vi "layout.vi"(0 "reference":refnum<class "SystemNode.lvclass">, 1 "graph":refnum<class "Graph.lvclass">, 2 "graphics":refnum<class "Graphics.lvclass">, 3 "grid":refnum<class "Grid.lvclass">, 5 "error in (no error)":errorcluster) -> (14 "reference out":refnum<class "SystemNode.lvclass">, 19 "error out":errorcluster)   [LabVIEW 2020, in "SystemNode.lvclass"]
doc: "public void draw(Graphics2D g2)"
uses:
  <resource>/Framework/Providers/Open_GDS/UML/SystemNode_class/SystemNode.lvclass
  C:/Program Files (x86)/National Instruments/LabVIEW 2020/resource/Framework/Providers/Open_GDS/UML/RectangularNode_class/RectangularNode.lvclass
  C:/Program Files (x86)/National Instruments/LabVIEW 2020/resource/Framework/Providers/Open_GDS/UML/AbstractNode_class/AbstractNode.lvclass
  <resource>/Framework/Providers/Open_GDS/UML/Grid_class/Grid.lvclass
  <resource>/Framework/Providers/Open_GDS/UML/Graphics_class/Graphics.lvclass
  <resource>/Framework/Providers/Open_GDS/UML/Graph_class/Graph.lvclass
  <resource>/Framework/Providers/Open_GDS/UML/General/Rectangle/Rectangle Rectangle2D.ctl
  <resource>/Framework/Providers/Open_GDS/UML/MultiLineString_class/MultiLineString.lvclass
  <resource>/Framework/Providers/Open_GDS/UML/AbstractNode_class/AbstractNode.lvclass
  <resource>/Framework/Providers/Open_GDS/UML/RectangularNode_class/RectangularNode.lvclass
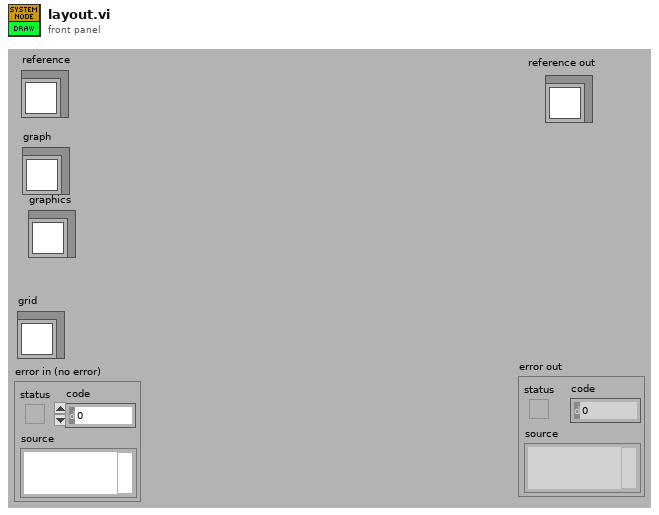
[diagram p1: front panel]
types:
  T1 = typedef "Rectangle Rectangle2D.ctl" = cluster{"x":dbl, "y":dbl, "width":dbl, "height":dbl}
  T2 = typedef "SystemNode.lvclass/ObjectAttributes.ctl" = cluster{"contents":refnum<class "MultiLineString.lvclass">, "DEFAULT_WIDTH":i32, "DEFAULT_HEIGHT":i32, "NAME_GAP":i32, "XGAP":i32, "YGAP":i32}
  T3 = typedef "RectangularNode.lvclass/ObjectAttributes.ctl" = cluster{"bounds":T1}
  T4 = typedef "AbstractNode.lvclass/ObjectAttributes.ctl" = cluster{"parent":refnum<class "AbstractNode.lvclass">, "children":refnum<class "AbstractNode.lvclass">[], "Hidden":bool}
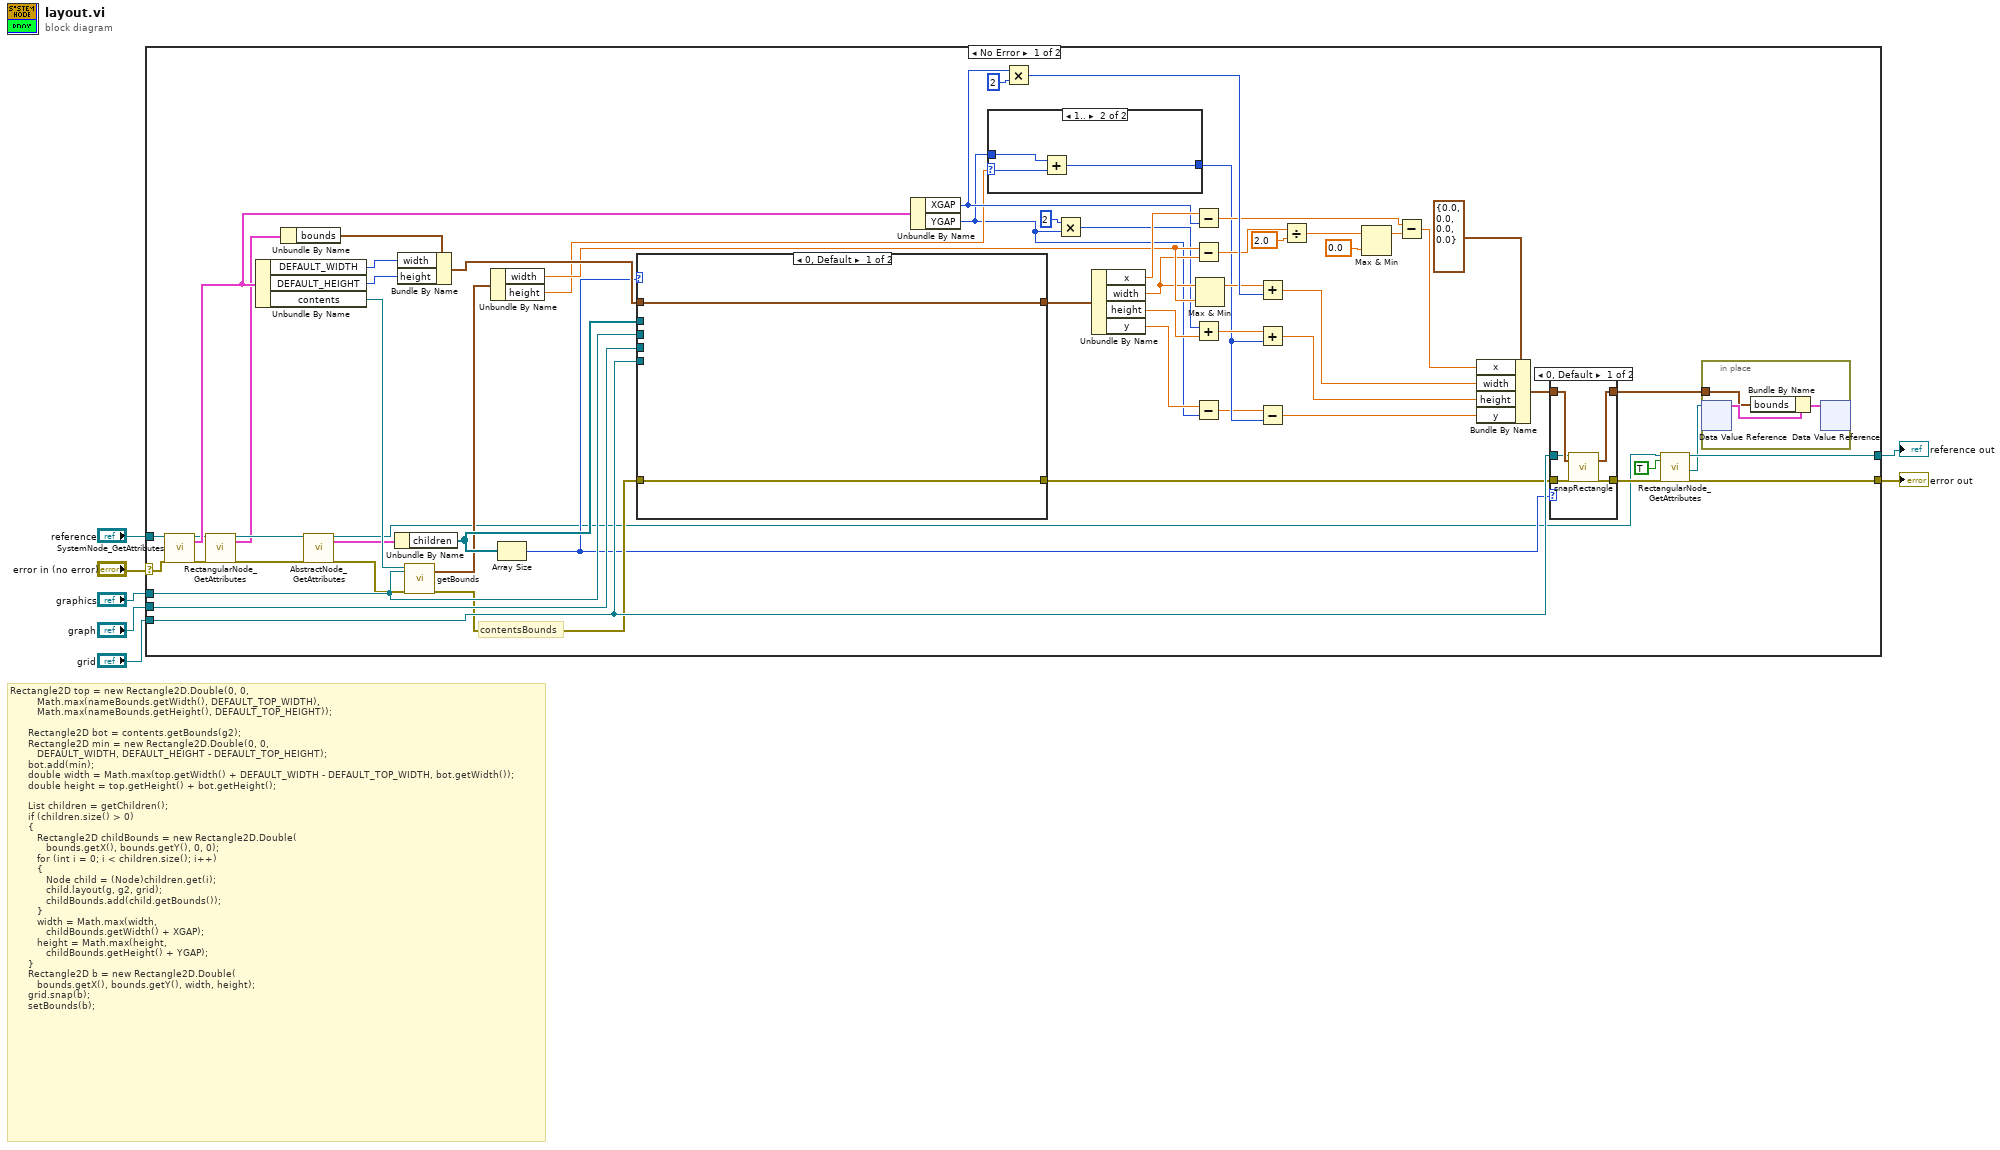
[diagram p0: block diagram]
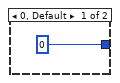
[diagram p3: hidden frame]
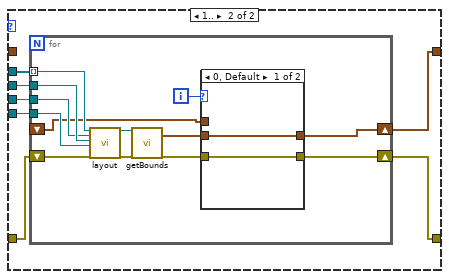
[diagram p4: hidden frame]
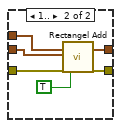
[diagram p5: hidden frame]
diagram:
  # "Rectangle2D top = new Rectangle2D.Double(0, 0,\n         Math.max(nameBounds.getWidth(), DEFAULT_TOP_WIDTH), \n         Math.max(nameBounds.getHeight(), DEFAULT_TOP_HEIGHT));\n\n      Rectangle2D bot = contents.getBounds(g2);\n      Rectangle2D min = new Rectangle2D.Double(0, 0,\n         DEFAULT_WIDTH, DEFAULT_HEIGHT - DEFAULT_TOP_HEIGHT);\n      bot.add(min);\n      double width = Math.max(top.getWidth() + DEFAULT_WIDTH - DEFAULT_TOP_WIDTH, bot.getWidth());\n      double height = top.getHeight() + bot.getHeight();\n\n      List children = getChildren();\n      if (children.size() > 0)\n      {\n         Rectangle2D childBounds = new Rectangle2D.Double(\n            bounds.getX(), bounds.getY(), 0, 0);\n         for (int i = 0; i < children.size(); i++)\n         {\n            Node child = (Node)children.get(i);\n            child.layout(g, g2, grid);\n            childBounds.add(child.getBounds());\n         }\n         width = Math.max(width, \n            childBounds.getWidth() + XGAP);\n         height = Math.max(height, \n            childBounds.getHeight() + YGAP);\n      }\n      Rectangle2D b = new Rectangle2D.Double(\n         bounds.getX(), bounds.getY(), width, height);\n      grid.snap(b);\n      setBounds(b);"
  n1 = case shown="No Error" "error in (no error)" {
    selector: "error in (no error)" -> [w63 w111]
    tunnel: "reference" -> [w66 w112]
    tunnel: [w65 w111] -> w6
    tunnel: [w64 w112] -> w5
    tunnel: "graphics" -> [w62 _]
    tunnel: "grid" -> [w61 _]
    tunnel: "graph" -> [w60 _]
    frame No Error {
      # "contentsBounds"
      n2 = call <resource>:"SystemNode_GetAttributes.vi"("reference in"=w66, "error in (no error)"=w63) -> ("reference out"=w17:refnum<class "SystemNode.lvclass">, "Data"=w18:T2, "error out"=w16:errorcluster)  [unwired: 1 in, 14 out]
      n3 = call <resource>:"RectangularNode_GetAttributes.vi"("reference in"=w17, "error in (no error)"=w16) -> ("reference out"=w15:refnum<class "SystemNode.lvclass">, "Data"=w10:T3, "error out"=w14:errorcluster)  [unwired: 14 in, 1 out]
      n4 = Unbundle By Name(w18) -> ("DEFAULT_WIDTH"=w56:i32, "DEFAULT_HEIGHT"=w57:i32, "contents"=w59:refnum<class "MultiLineString.lvclass">)
      n5 = Unbundle By Name(w10) -> ("bounds"=w55:T1)
      n6 = call <resource>:"AbstractNode_GetAttributes.vi"("reference in"=w15, "error in (no error)"=w14) -> ("reference out"=w12:refnum<class "SystemNode.lvclass">, "Data"=w11:T4, "error out"=w13:errorcluster)  [unwired: 14 in, 1 out]
      n7 = Unbundle By Name(w11) -> ("children"=w58:refnum<class "AbstractNode.lvclass">[])
      n8 = Bundle By Name(cluster=w55, "width"=w56, "height"=w57) -> (w53:T1)
      n9 = call-dynamic "getBounds.vi"("reference"=w59, "graphics"=w62, "error in (no error)"=w13) -> ("bounds"=w45:T1, "error out"=w54:errorcluster)  [unwired: 14 in, 1 out]
      n10 = Unbundle By Name(w45) -> ("width"=w43:dbl, "height"=w28:dbl)
      n11 = Array Size(array=w58) -> (size(s)=w20:i32)
      n12 = case shown="0, Default" w20 {
        tunnel: w54 -> [w82 w89]
        tunnel: w58 -> [_ w88]
        tunnel: w53 -> [w81 _]
        tunnel: [w82 w83] -> w21
        tunnel: w61 -> [_ w87]
        tunnel: w62 -> [_ w86]
        tunnel: w60 -> [_ w85]
        tunnel: [w81 w84] -> w50
        frame 0, Default {
        }
        frame 1.. {
          n13 = for {
            tunnel: w88 -> [w100] mode=indexing
            shift-right: [w102] -> w83
            shift-left: w89 -> [w101]
            shift-right: [w96] -> w84
            shift-left: _ -> [w92]
            tunnel: w87 -> [w95]
            tunnel: w86 -> [w94]
            tunnel: w85 -> [w93]
            i -> [w90]
            n14 = call-dynamic "layout.vi"("reference"=w100, "graph"=w93, "graphics"=w94, "grid"=w95, "error in (no error)"=w101) -> ("reference out"=w99:refnum<class "AbstractNode.lvclass">, "error out"=w98:errorcluster)  [unwired: 13 in]
            n15 = call-dynamic "getBounds.vi"("reference"=w99, "error in (no error)"=w98) -> ("bounds"=w91:T1, "error out"=w97:errorcluster)  [unwired: 15 in, 1 out]
            n16 = case shown="0, Default" w90 {
              tunnel: [w104 w110] -> w102
              tunnel: w97 -> [w104 w109]
              tunnel: [w103 w108] -> w96
              tunnel: w92 -> [_ w107]
              tunnel: w91 -> [w103 w106]
              frame 0, Default {
              }
              frame 1.. {
                n17 = call <resource>:"Rectangel Add.vi"("bounds1"=w107, "bounds2"=w106, "error in (no error)"=w109, "useAbsoluteCordinates(False)"=TRUE) -> ("boundsAdded"=w108:T1, "error out"=w110:errorcluster)  [unwired: 1 in, 13 out]
              }
            }
          }
        }
      }
      n18 = Unbundle By Name(w18) -> ("XGAP"=w46:i32, "YGAP"=w24:i32)
      n19 = case shown="1.." w28 {
        selector: w28 -> [_ w80]
        tunnel: w24 -> [_ w79]
        tunnel: [0 w78] -> w27
        frame 0, Default {
        }
        frame 1.. {
          n20 = Add(x=w79, y=w80) -> (x+y=w78:i32)
        }
      }
      n21 = Multiply(x=w46, y=2) -> (x*y=w48:i32)
      n22 = Multiply(x=2, y=w24) -> (x*y=w32:i32)
      n23 = Unbundle By Name(w50) -> ("x"=w49:dbl, "width"=w42:dbl, "height"=w33:dbl, "y"=w25:dbl)
      n24 = Subtract(x=w49, y=w46) -> (x-y=w40:dbl)
      n25 = Subtract(x=w43, y=w42) -> (x-y=w39:dbl)
      n26 = Add(x=w32, y=w33) -> (x+y=w30:dbl)
      n27 = Subtract(x=w25, y=w24) -> (x-y=w26:dbl)
      n28 = Max & Min(x=w42, y=w43) -> (max(x,y)=w44:dbl)  [unwired: 1 out]
      n29 = Add(x=w44, y=w48) -> (x+y=w47:dbl)
      n30 = Add(x=w30, y=w27) -> (x+y=w29:dbl)
      n31 = Subtract(x=w26, y=w27) -> (x-y=w34:dbl)
      n32 = Divide(x=w39, y=2.0) -> (x/y=w37:dbl)
      n33 = Max & Min(x=w37, y=0.0) -> (max(x,y)=w35:dbl)  [unwired: 1 out]
      n34 = Subtract(x=w40, y=w35) -> (x-y=w41:dbl)
      n35 = Bundle By Name(cluster=T1 {"x"=0.0, "y"=0.0, "width"=0.0, "height"=0.0} ("input cluster"), "x"=w41, "width"=w47, "height"=w29, "y"=w34) -> (w23:T1)
      n36 = case shown="0, Default" w20 {
        tunnel: w23 -> [w74 w75]
        tunnel: [w73 w75] -> w8
        tunnel: [w72 w76] -> w22
        tunnel: w21 -> [w71 w76]
        tunnel: w61 -> [w70 _]
        frame 0, Default {
          n37 = call <resource>:"snapRectangle.vi"("reference"=w70, "bounds"=w74, "error in (no error)"=w71) -> ("boundsOut"=w73:T1, "error out"=w72:errorcluster)  [unwired: 15 out]
        }
        frame 1.. {
        }
      }
      n38 = call <resource>:"RectangularNode_GetAttributes.vi"("reference in"=w12, "OnlyGetDvrReference(False)"=TRUE, "error in (no error)"=w22) -> ("reference out"=w64:refnum<class "SystemNode.lvclass">, "DataRef"=w9:refnum<data-value>, "error out"=w65:errorcluster)  [unwired: 13 in, 1 out]
      n39 = in-place {
        in-place-border: w8 -> [w68]
        n40 = in-place-dvr #1(w9) -> (w69:T3)  [unwired: 1 out]
        n41 = Bundle By Name(cluster=w69, "bounds"=w68) -> (w67:T3)
        n42 = in-place-dvr #1(w67) -> ()  [unwired: 2 out]
      }
    }
    frame Error {
    }
  }
  "reference out" <- w5
  "error out" <- w6
